vi "Test Get Main Menu.vi"() -> ()   [LabVIEW 2026]
doc: "Caraya unit test for Get Main Menu.vi (feature #47: Fast Cash $100 replaces the reserved None item).\n\nGet Main Menu.vi is called once. The expected menu is ONE constant, an instance of the typedef ATM Menu.ctl, so it follows the typedef when the states enum grows. Do not replace it with an unlinked copy: Caraya compares the enum's item list too. The expected value of a single item is unbundled from that same constant.\n\nRow 1: the top left item (Left, Item 1) is labelled Fast Cash $100 and its action is the state Fast Cash $100.\nRow 2: the bottom right item (Right, Item 3) is still labelled Fast Cash $50 and its action is still the state Fast Cash.\nRow 3: the whole menu equals the specified six items, none of which has the action None any more.\n\nEvery assertion takes its error in from Define Test rather than from the assertion before it, so a failing row cannot stop a later one. The error cluster carries the FIRST failure only. Read the JUnit report for all of them."
uses:
  <vilib>/addons/_JKI Toolkits/Caraya/classes/Test/Test.lvclass
  <vilib>/addons/_JKI Toolkits/Caraya/classes/Assert/Assert.lvclass
  Controls/ATM States.ctl
  Controls/ATM Menu Item.ctl
  Controls/ATM Menu Side.ctl
  Controls/ATM Menu.ctl
panel:
  out "error out":errorcluster
  in  "error in":errorcluster
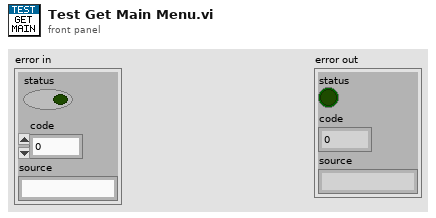
[diagram p1: front panel]
types:
  T1 = typedef "ATM Menu.ctl" = cluster{"Left":T2, "Right":T2}
  T2 = typedef "ATM Menu Side.ctl" = cluster{"Item 1":T3, "Item 2":T3, "Item 3":T3}
  T3 = typedef "ATM Menu Item.ctl" = cluster{"Label":string, "Action":T4}
  T4 = typedef "ATM States.ctl" = enum16{"Initialize", "Wait for Event", "Card Inserted", "Process Input", "Verify Account", "Show Main Menu", "Deposit Prompt", "Withdraw Prompt", "Deposit", "Withdraw", "Fast Cash", "Balance Inquiry", "None", "Terminate Session", "Exit", "Fast Cash $100"}
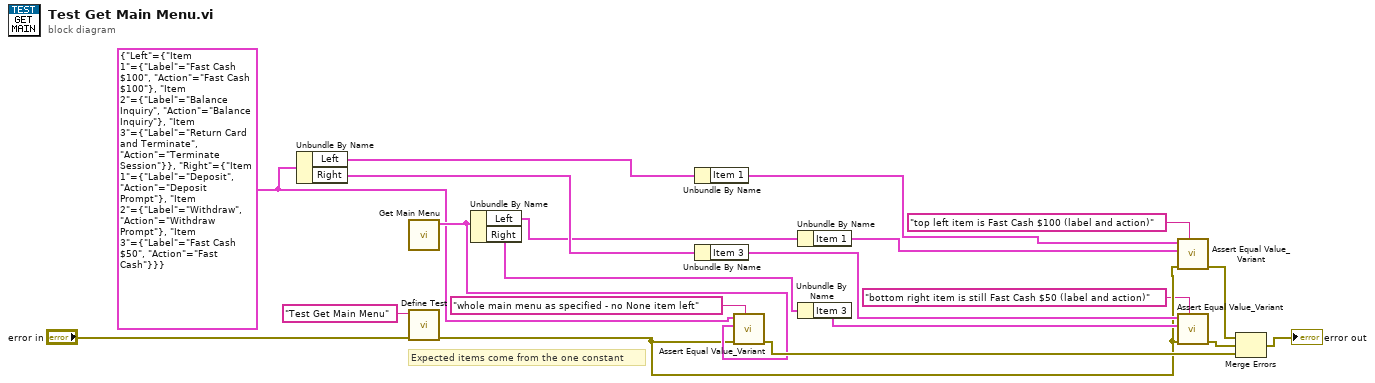
[diagram p0: block diagram]
diagram:
  w4 = T1 {"Left"={"Item 1"={"Label"="Fast Cash $100", "Action"=enum."Fast Cash $100"}, "Item 2"={"Label"="Balance Inquiry", "Action"=enum."Balance Inquiry"}, "Item 3"={"Label"="Return Card and Terminate", "Action"=enum."Terminate Session"}}, "Right"={"Item 1"={"Label"="Deposit", "Action"=enum."Deposit Prompt"}, "Item 2"={"Label"="Withdraw", "Action"=enum."Withdraw Prompt"}, "Item 3"={"Label"="Fast Cash $50", "Action"=enum."Fast Cash"}}} ("expected Main Menu")
  # "Expected items come from the one constant"
  n1 = Unbundle By Name(w4) -> ("Left"=w14:T2, "Right"=w15:T2)
  n2 = call "Get Main Menu.vi"() -> ("Main Menu"=w9:T1)  [unwired: 10 in, 1 out]
  n3 = call <vilib>:"Define Test.vi"("error in (no error)"="error in", "Label (VI Title)"="Test Get Main Menu") -> ("error out"=w8:errorcluster)  [unwired: 8 in, 1 out]
  n4 = Unbundle By Name(w9) -> ("Left"=w10:T2, "Right"=w11:T2)
  n5 = Unbundle By Name(w14) -> ("Item 1"=w16:T3)
  n6 = Unbundle By Name(w15) -> ("Item 3"=w17:T3)
  n7 = call <vilib>:"Assert Equal Value_Variant.vi"("Label"="whole main menu as specified - no None item left" ("Label 3"), "error in (no error)"=w8, "Actual"=w9, "Expected"=w4) -> ("error out"=w20:errorcluster)  [unwired: 6 in, 1 out]
  n8 = Unbundle By Name(w10) -> ("Item 1"=w12:T3)
  n9 = Unbundle By Name(w11) -> ("Item 3"=w13:T3)
  n10 = call <vilib>:"Assert Equal Value_Variant.vi"("Label"="top left item is Fast Cash $100 (label and action)" ("Label 1"), "error in (no error)"=w8, "Actual"=w12, "Expected"=w16) -> ("error out"=w18:errorcluster)  [unwired: 6 in, 1 out]
  n11 = call <vilib>:"Assert Equal Value_Variant.vi"("Label"="bottom right item is still Fast Cash $50 (label and action)" ("Label 2"), "error in (no error)"=w8, "Actual"=w13, "Expected"=w17) -> ("error out"=w19:errorcluster)  [unwired: 6 in, 1 out]
  n12 = Merge Errors(w18, w19, w20) -> (→"error out":errorcluster)
